vi "turn on off Keysight 9020A Correction Factor.vi"(8 "error in (no error)":errorcluster, 9 "Correction Applied?":bool, 10 "Target Correction Table":T1(ring), 11 "FSV-40N in":refnum<class "FSV-40N.lvclass">) -> (0 "error out":errorcluster, 3 "FSV-40N out":refnum<class "FSV-40N.lvclass">)   [LabVIEW 2023, in "Spectrum Analyzer.lvlib" / "FSV-40N.lvclass"]
uses:
  FSV-40N.lvclass
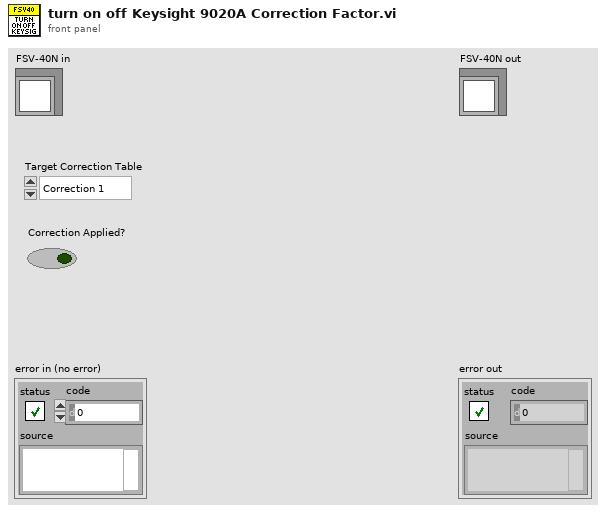
[diagram p1: front panel]
types:
  T1 = enum16{"Correction 1", "Correction 2", "Correction 3", "Correction 4", "Correction 5", "Correction 6", "Correction 7", "Correction 8"}
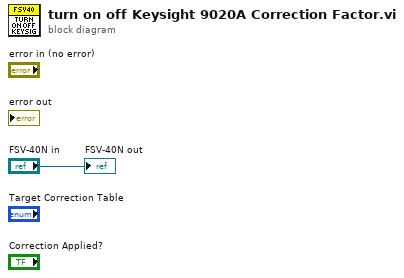
[diagram p0: block diagram]
diagram:
  "FSV-40N out" <- "FSV-40N in"
